vi "Add.vi"(6 "Options":T1={"DbType"=-1, "Direction"=-1, "Size"=-1, "Precision"=255, "Scale"=255} {"Direction" items=["Input"=1, "Output"=2, "InputOutput"=3, "ReturnValue"=6]; "DbType" items=["AnsiString"=0, "Binary"=1, "Byte"=2, "Boolean"=3, "Currency"=4, "Date"=5, "DateTime"=6, "Decimal"=7, "Double"=8, "Guid"=9, "Int16"=10, "Int32"=11, "Int64"=12, "Object"=13, "SByte"=14, "Single"=15, "String"=16, "Time"=17, "UInt16"=18, "UInt32"=19, "UInt64"=20, "VarNumeric"=21, "AnsiStringFixedLength"=22, "StringFixedLength"=23, "Xml"=25, "DateTime2"=26, "DateTimeOffset"=27]}, 8 "error in (no error)":errorcluster, 9 "value":variant, 10 "name":string, 11 "PGJDPParameter in":refnum<class "Parameter.lvclass">) -> (0 "error out":errorcluster, 3 "PGJDPParameter out":refnum<class "Parameter.lvclass">)   [LabVIEW 2020, in "ORM_pgsql_jdp.lvlib" / "Parameter.lvclass"]
uses:
  Parameter.lvclass
  C:/Program Files/National Instruments/LabVIEW 2020/vi.lib/Viviota/shared/ORM.lvlibp/DynamicParameters/DynamicParameters.lvclass
  <vilib>/Viviota/shared/ORM.lvlibp/DynamicParameters/Read ParameterNames.vi
  <vilib>/Viviota/shared/ORM.lvlibp/DynamicParameters/DynamicParameters.lvclass
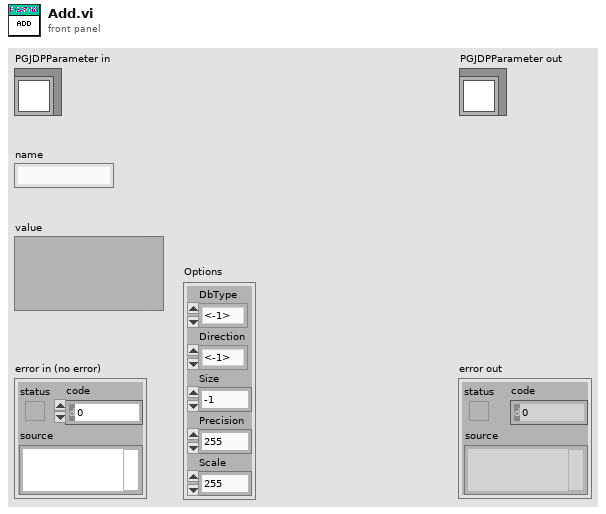
[diagram p1: front panel]
types:
  T1 = cluster{"DbType":i32, "Direction":i32, "Size":i32, "Precision":u8, "Scale":u8}
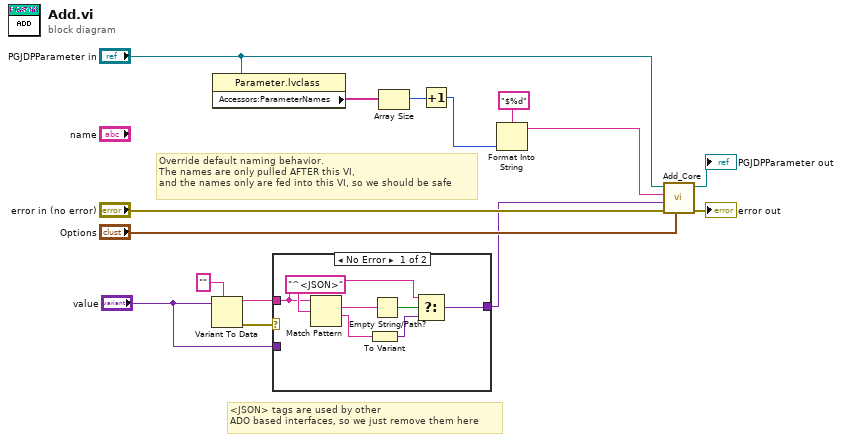
[diagram p0: block diagram]
diagram:
  # "<JSON> tags are used by other\nADO based interfaces, so we just remove them here"
  # "Override default naming behavior.\nThe names are only pulled AFTER this VI, \nand the names only are fed into this VI, so we should be safe"
  n1 = Variant To Data(type="", Variant="value") -> (data=w3:string, error out=w4:errorcluster)  [unwired: 1 in]
  n2 = property class="Parameter.lvclass"(reference="PGJDPParameter in") -> ("Accessors:ParameterNames"=w10:string[])  [unwired: 1 in, 2 out]
  n3 = case shown="No Error" w4 {
    tunnel: w3 -> [w19 _]
    tunnel: [w16 w23] -> w1
    tunnel: "value" -> [_ w23]
    frame No Error {
      n4 = Match Pattern(string=w19, regular expression="^<JSON>") -> (match substring=w20:string, after substring=w18:string)  [unwired: 1 in, 2 out]
      n5 = To Variant(anything=w18) -> (Variant=w17:variant)
      n6 = Empty String/Path?(string/path=w20) -> (empty?=w21:bool)
      n7 = Select(t=w19, s=w21, f=w17) -> (s? t:f=w16:variant)
    }
    frame Error {
    }
  }
  n8 = Array Size(array=w10) -> (size(s)=w9:i32)
  n9 = Increment(x=w9) -> (x+1=w8:i32)
  n10 = Format Into String(format string="$%d", w8) -> (resulting string=w6:string)  [unwired: 2 in, 1 out]
  n11 = call <vilib>:"Add_Core.vi"("Options"="Options", "error in (no error)"="error in (no error)", "value"=w1, "name"=w6, "DynamicParameters in"="PGJDPParameter in") -> ("error out"=→"error out":errorcluster, "DynamicParameters out"=→"PGJDPParameter out":refnum<class "Parameter.lvclass">)  [unwired: 5 in]
